vi "Write.vi"(5 "Username":string, 6 "Password":string, 7 "Address":string, 8 "Error In":errorcluster) -> (0 "Error Out":errorcluster)   [LabVIEW 2018, in "Tests.lvlib" / "SFTP File.lvlib"]
uses:
  SFTP File.lvlib
  src/Toolkit/SFTP File/Type Definitions/Open Options.ctl
  src/Toolkit/SFTP File/Support/Open from SFTP.vi
  src/Toolkit/SFTP File/Support/Close to SFTP.vi
  <vilib>/addons/_JKI Toolkits/Caraya/classes/Test/Test.lvclass
  <vilib>/addons/_JKI Toolkits/Caraya/classes/Assert/Assert.lvclass
  src/Toolkit/SFTP File/SFTP File.lvclass
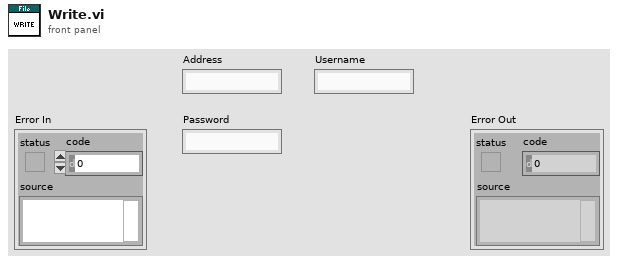
[diagram p1: front panel]
types:
  T1 = typedef "Toolkit.lvlib/SFTP File.lvclass/Open Options.ctl" = cluster{"Read":bool, "Write":bool, "Append":bool, "Create":bool, "Truncate":bool, "Exclude":bool}
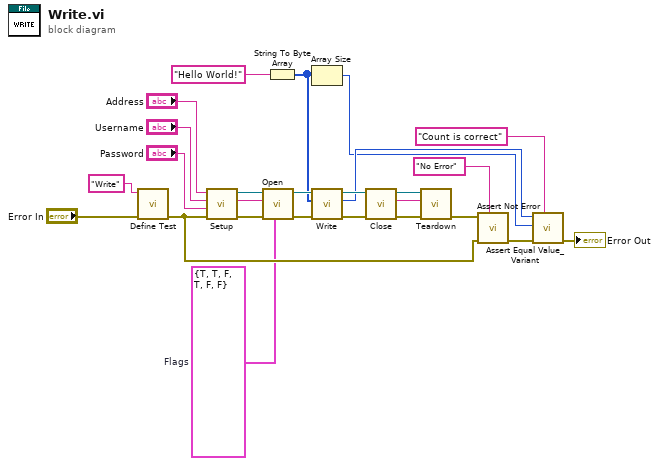
[diagram p0: block diagram]
diagram:
  w6 = T1 {"Read"=TRUE, "Write"=TRUE, "Append"=FALSE, "Create"=TRUE, "Truncate"=FALSE, "Exclude"=FALSE}  # Flags
  n1 = call <vilib>:"Define Test.vi"("error in (no error)"="Error In", "Label (VI Title)"="Write") -> ("error out"=w17:errorcluster)  [unwired: 9 in]
  n2 = call "Setup.vi"("Error In"=w17, "Password"="Password", "Username"="Username", "Address"="Address") -> ("Error Out"=w4:errorcluster, "Temporary File"=w5:string, "SFTP"=w15:refnum<class "SFTP.lvclass">)  [unwired: 5 in]
  n3 = call-poly "Open.vi"("Options"=w6, "Error In"=w4, "Remote Path"=w5, "SFTP"=w15) -> ("Error Out"=w10:errorcluster, "SFTP File"=w14:refnum<class "SFTP File.lvclass">)  [unwired: 6 in]
  n4 = String To Byte Array(string="Hello World!") -> (unsigned byte array=w8:u8[])
  n5 = Array Size(array=w8) -> (size(s)=w7:i32)
  n6 = call "Write.vi"("Error In"=w10, "Data"=w8, "SFTP File In"=w14) -> ("Error Out"=w12:errorcluster, "Count"=w11:i64, "SFTP File Out"=w13:refnum<class "SFTP File.lvclass">)  [unwired: 6 in]
  n7 = call-poly "Close.vi"("Error In"=w12, "SFTP File"=w13) -> ("Error Out"=w1:errorcluster, "Remote Path"=w3:string, "SFTP"=w2:refnum<class "SFTP.lvclass">)  [unwired: 7 in]
  n8 = call "Teardown.vi"("Error In"=w1, "Temporary File"=w3, "SFTP"=w2) -> ("Error Out"=w16:errorcluster)  [unwired: 8 in]
  n9 = call <vilib>:"Assert Not Error.vi"("Label"="No Error", "error in (no error)"=w17, "Not Error?"=w16) -> ("error out"=w23:errorcluster)  [unwired: 8 in]
  n10 = call <vilib>:"Assert Equal Value_Variant.vi"("Label"="Count is correct", "error in (no error)"=w23, "Y"=w7, "X"=w11) -> ("error out"=→"Error Out":errorcluster)  [unwired: 7 in]
